vi "Receiver_Example - 2 Channel - Experiment_17.vi"() -> ()   [LabVIEW 2022 SP3]
panel:
  out "SNR dB LP":dbl
  out "SNR dB HP":dbl
  out "size(s) 4":i32
  out "size(s) 3":i32
  out "size(s) 2":i32
  out "x*y":i32
  out "Payload_LP":i32=720
  out "Payload_HP":i32=720
  out "size(s)":i32
  in  "stop":bool
  out "BER LP3":dbl
  out "BER HP3":dbl
  out "Inst. BER LP - CH1":dbl format="%#_4g"
  out "OutputHPCH0":i8[](array[numeric])
  out "BER 16QAM":dbl
  out "LP - CH0":dbl format="%#_4g"
  out "Numeric":i32
  out "HP - CH0":dbl format="%#_4g"
  out "x = 0?":bool
  out "iterationsIM":dbl
  in  "State":i32
  in  "Counter":dbl
  in  "Tab Control 3":enum32{"OFDM - 4QAM", "16QAM"}(tab)
  in  "Switch mode":bool
  in  "Tab Control":T1(tab)
  in  "USRP ControledParameters":T2={"Active Antenna"="RX2", "Gain (dB)"=20.0, "Carrier Frequency"=2400000000.0, "IQ Rate"=2000000.0, "Active channels"="0,1"} {"IQ Rate" format="%#_6p"; "Carrier Frequency" format="%#_6p"; "Gain (dB)" format="%#_6f"}
  in  "Device selection":refnum<k15>="RIO0"
  in  "Trigger level":dbl=0.01 format="%f"
  out "CH0 - HP":T3
  out "CH1 - HP":T3
  out "SIG valid? - CH1":bool
  out "SIG valid? - CH0":bool
  out "Frequency offset - CH1":dbl
  out "Frequency offset - CH0":dbl
  out "Coerced Parameters":T4={"IQ Rate"=100000.0, "Carrier  Freq."=100000.0, "Gain"=0.0} {"Gain" format="%#_6f"; "Carrier  Freq." format="%#_6p"; "IQ Rate" format="%#_6p"}
  out "Error out":errorcluster
  out "CH0 - LP":T3
  out "CH1 - LP":T3
  out "Inst. BER HP - CH0":dbl format="%#_4g"
  out "Acc. BER HP - CH0":dbl format="%#_4g"
  out "Acum. Err HP - CH0":dbl
  out "No. Bits HP - CH0":dbl
  out "Acc. BER LP - CH0":dbl format="%#_4g"
  out "Inst. BER - CH1":dbl format="%#_4g"
  out "Inst. BER LP - CH0":dbl format="%#_4g"
  out "No. Bits - CH1":dbl
  out "No. Bits LP - CH0":dbl
  out "Acum. Err - CH1":dbl
  out "Acum. Err LP - CH0":dbl
  in  "Record BER":bool
  in  "Refresh Button":bool
  out "Acc. BER - CH1":dbl format="%#_4g"
  in  "Boolean 2":bool
  in  "Expected message HP - CH0":string="Critical Dataaaaa\nCritical Dataaaaa\nCritical Dataaaaa\nCritical Dataaaaa\nCritical Dataaaaa"
  out "Expected message HP Detected CH0":string="Non Critical Data\nNon Critical Data\nNon Critical Data\nNon Critical Data\nNon Critical Data"
  in  "Boolean 3":bool
  in  "Boolean":bool
  out "Expected message HP Detected CH1":string="Non Critical Data\nNon Critical Data\nNon Critical Data\nNon Critical Data\nNon Critical Data"
  out "Expected message LP Detected CH0":string="Non Critical Data\nNon Critical Data\nNon Critical Data\nNon Critical Data\nNon Critical Data"
  in  "Expected message - CH1":string="Critical Dataaaaa\nCritical Dataaaaa\nCritical Dataaaaa\nCritical Dataaaaa\nCritical Dataaaaa"
  in  "Expected message LP - CH0":string="Non Critical Data\nNon Critical Data\nNon Critical Data\nNon Critical Data\nNon Critical Data"
  in  "Boolean 5":bool
  in  "Expected message LP - CH1":string="Non Critical Data\nNon Critical Data\nNon Critical Data\nNon Critical Data\nNon Critical Data"
  out "Expected message LP Detected CH1":string="Non Critical Data\nNon Critical Data\nNon Critical Data\nNon Critical Data\nNon Critical Data"
  in  "High-Power Window Size":dbl=15.0 format="%#_6p"
  in  "Low-Power Window Size - CH0":dbl=15.0 format="%#_6p"
  in  "Channel":bool
  in  "Expected message HP - CH0 2":string="Critical Dataaaaa\nCritical Dataaaaa\nCritical Dataaaaa\nCritical Dataaaaa\nCritical Dataaaaa\nNon Critical Data\nNon Critical Data\nNon Critical Data\nNon Critical Data\nNon Critical Data"
  in  "Tab Control 2":enum32{"1 Channel", "2 Channel"}(tab)
  in  "Save data 1 channel":bool
  out "Constellation Map 1 Channel":cdb[](graph)
  out "Low-Power BER - 1 Channel":dbl(graph)
  out "High-Power BER - 1 Channel":dbl(graph)
  out "High-Power Decoded message - 1 Channel":string
  out "Low-Power Decoded message - 1 Channel":string
  out "Low-Power Decoded message - CH0":string
  out "Decoded message - CH1":string
  out "Constellation Map 2 Channel":cluster{"Constellation":cdb[]}[](graph)
  out "Low-Power BER - 2 Channels":T5(graph)
  out "High-Power BER":T6(graph)
  out "High-Power Decoded message - CH0":string
  out "Low-Power Decoded message - CH1":string
  out "CH1 2":bool
  out "CH0 2":bool
  in  "Save data 2 channels":bool
  in  "Color Box 3":u32(colorbox)=11025761
  in  "Color Box 4":u32(colorbox)=7377308
  out "SNR dB":dbl
  in  "Save data":bool
  out "Expected message  HP  Detected 2":string="Critical Dataaaaa\nCritical Dataaaaa\nCritical Dataaaaa\nCritical Dataaaaa\nCritical Dataaaaa"
  in  "Boolean 4":bool
  in  "High-Power Window Size 2":dbl=15.0 format="%#_6p"
  out "High-Power Instantaneous BER Graph 2":u8(slide) scale=0.0..100.0
  out "High-Power BER Graph 2":dbl(graph)
  out "No. Bits HP 2":dbl
  out "Acc. BER  HP 2":dbl format="%#_4g"
  out "Acum. Err HP 2":dbl
  out "Inst. BER HP 2":dbl format="%#_4g"
  in  "Expected message 2 HP 2":string="Critical Dataaaaa\nCritical Dataaaaa\nCritical Dataaaaa\nCritical Dataaaaa\nCritical Dataaaaa"
  out "High-Power Decoded Message 2":string
  in  "Record BER 2":bool
  out "Constellation Map 2":cdb[](graph)
  out "Frequency offset 2":dbl
  out "SIG valid? 2":bool
  in  "Refresh Button 2":bool
  out "Error out 2":errorcluster
  in  "error in (no error)":errorcluster
  # "OFDM Superposition Coded Receiver"
  # "Superposition coded\n(criticality-aware)"
  # "Single stream\n(criticality-agnostic)"
  # "1 Channel"
  # "2 Channel"
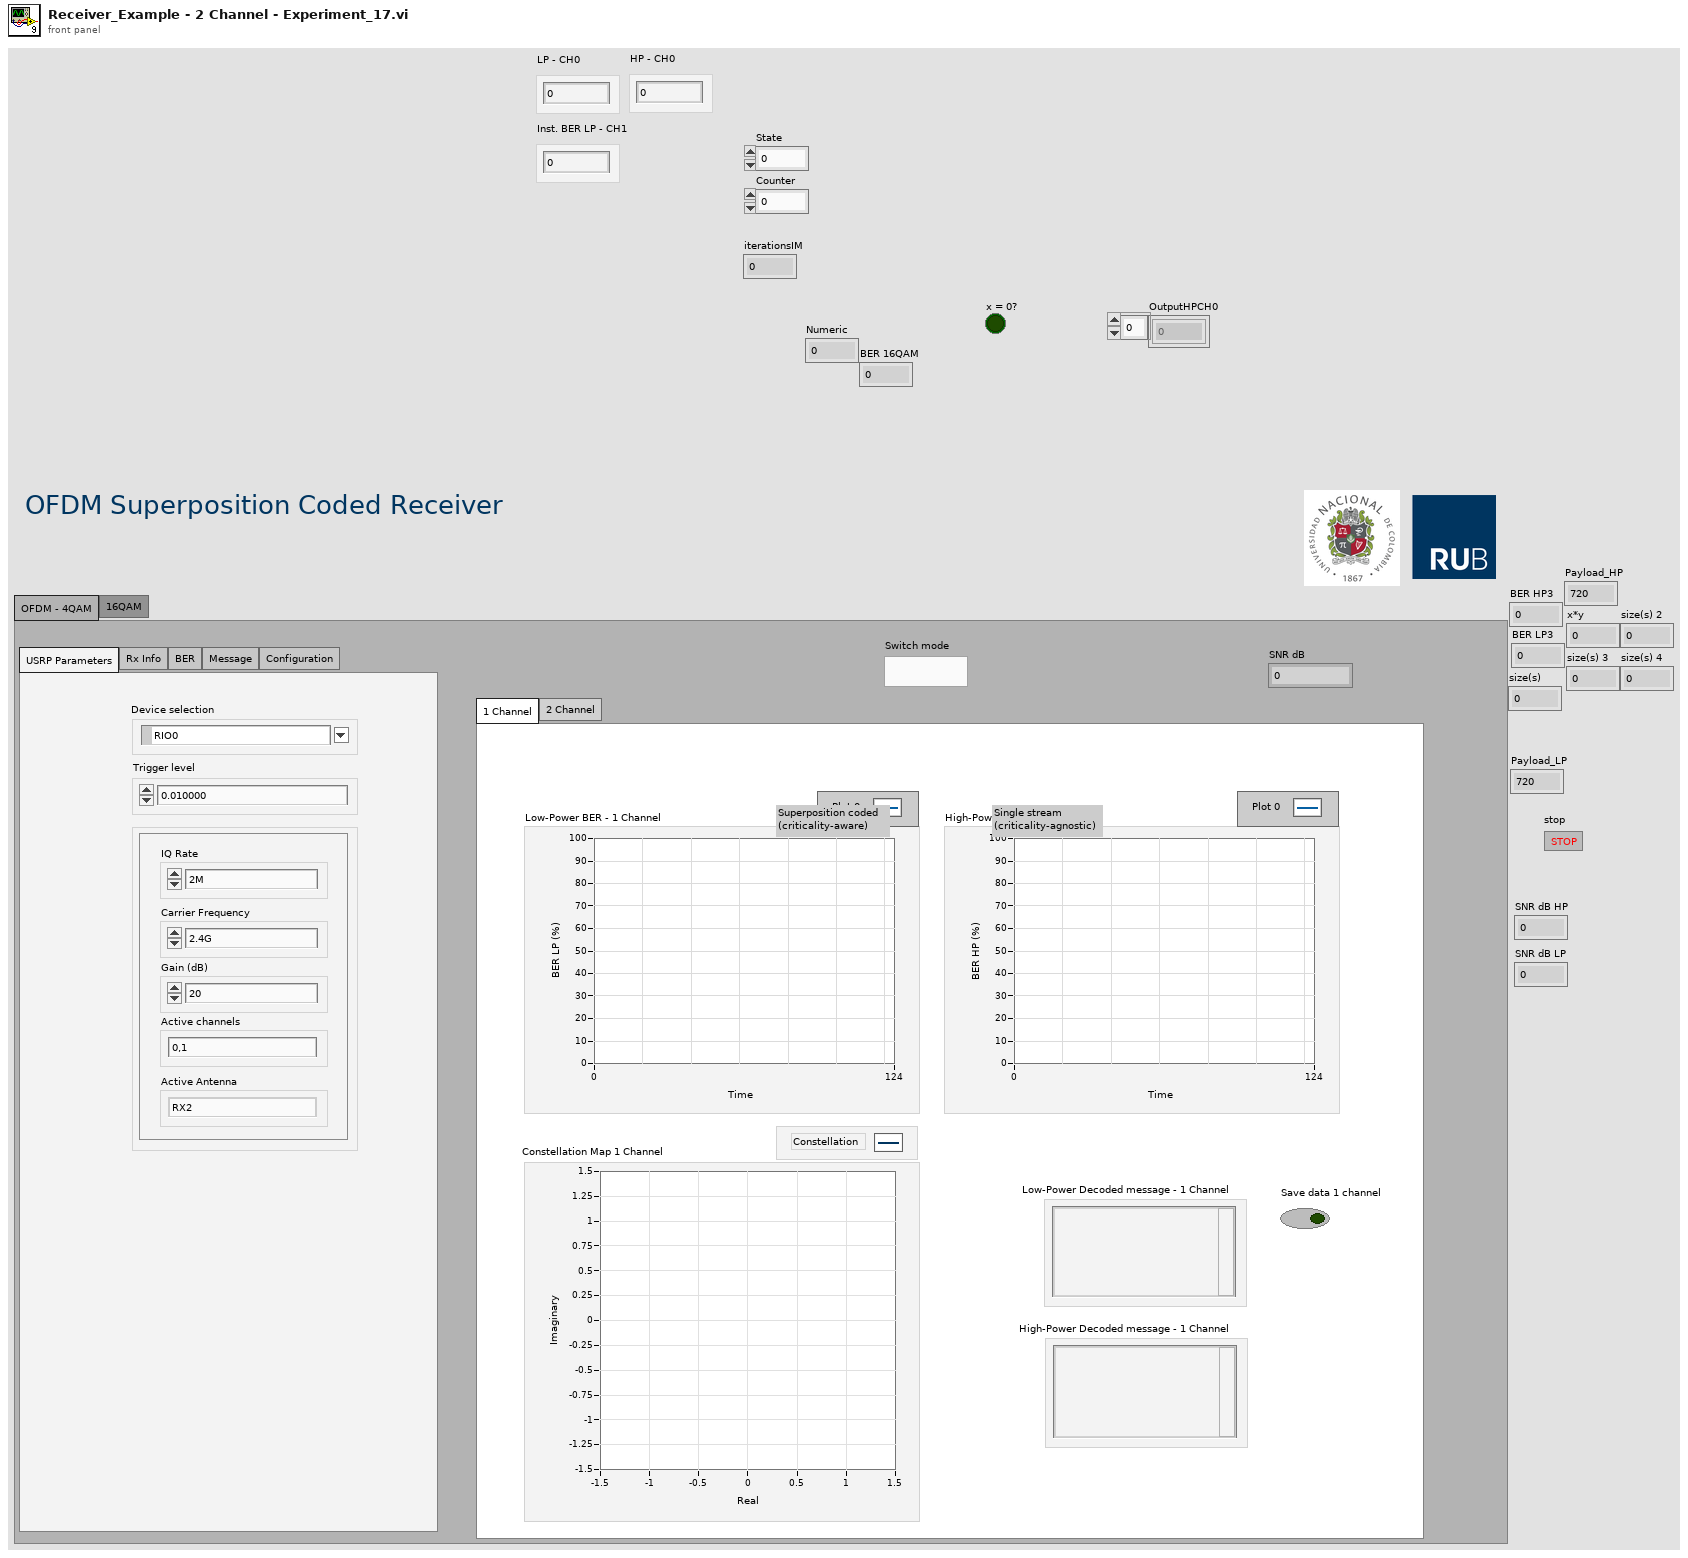
[diagram p1: front panel]
types:
  T1 = enum32{"USRP Parameters", "Rx Info", "BER", "Message", "Configuration"}
  T2 = cluster{"Active Antenna":string, "Gain (dB)":dbl, "Carrier Frequency":dbl, "IQ Rate":dbl, "Active channels":string}
  T3 = cluster{"Modulation type":enum16{"QPSK(4QAM)", "64QAM", "16QAM", "BPSK"}, "BCC rate (k/n)":enum16{"1/2", "2/3", "3/4"}}
  T4 = cluster{"IQ Rate":dbl, "Carrier  Freq.":dbl, "Gain":dbl}
  T5 = cluster{"Graph Instantaneous BER":dbl, "Graph Instantaneous BER":dbl, "Graph Instantaneous BER":dbl}
  T6 = cluster{"Graph Instantaneous BER":dbl, "Graph Instantaneous BER":dbl, "Inst. BER - CH1":dbl}
  T7 = enum16{"open", "replace", "create", "open or create", "replace or create", "replace or create with confirmation"}
  T8 = cluster{"coerced IQ rate":dbl, "coerced carrier frequency":dbl, "coerced gain":dbl}
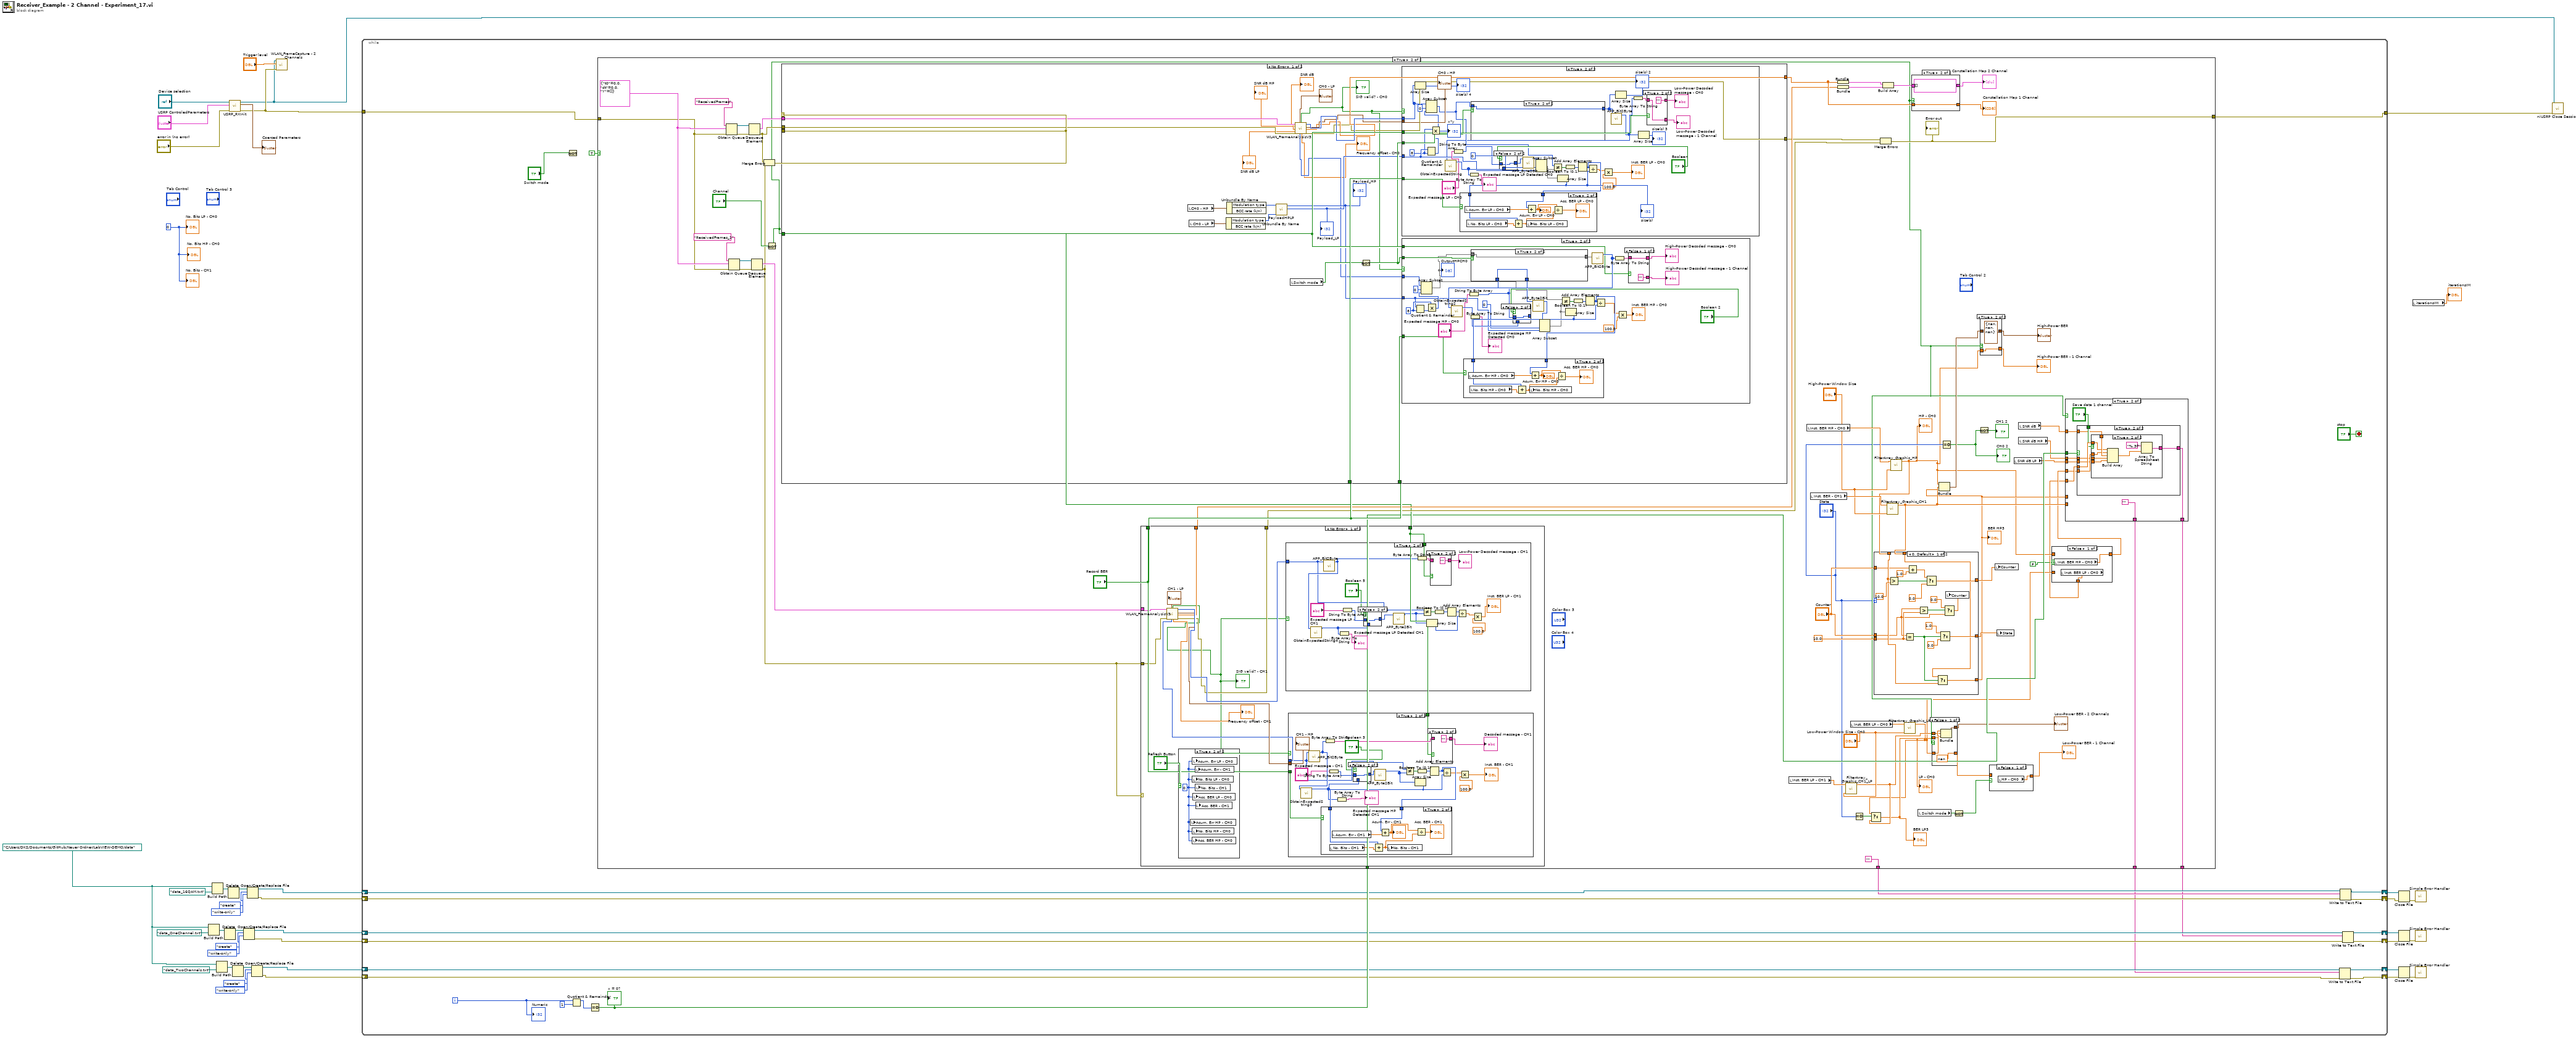
[diagram p0: block diagram]
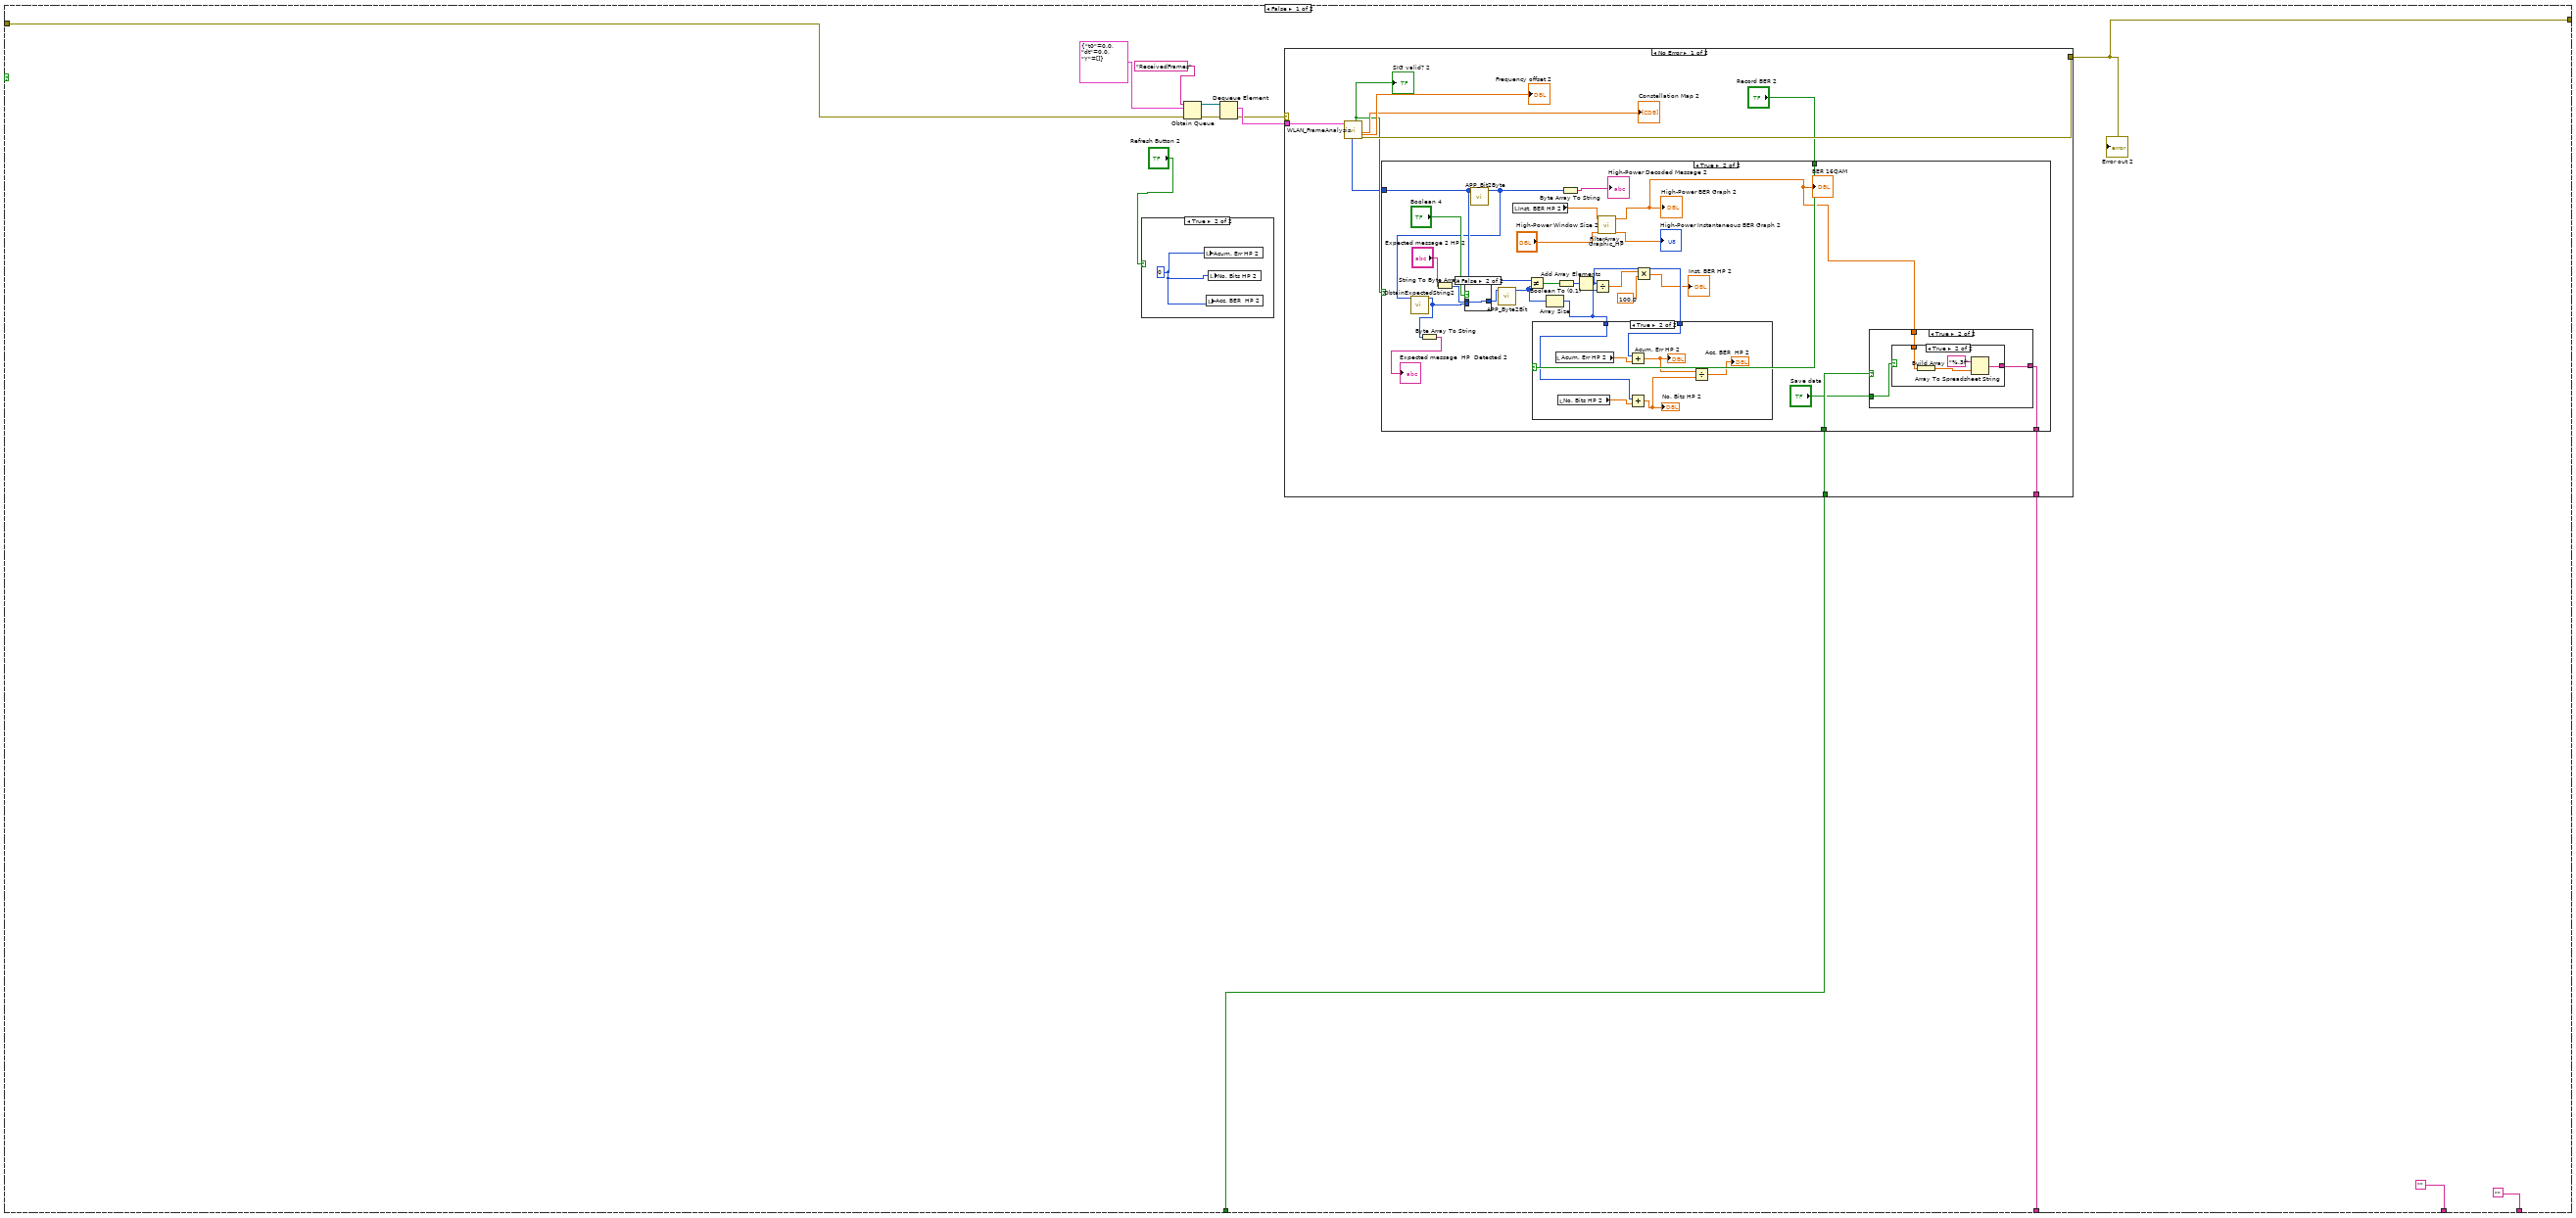
[diagram p2: hidden frame]
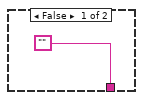
[diagram p4: hidden frame]
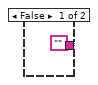
[diagram p5: hidden frame]
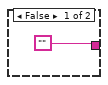
[diagram p6: hidden frame]
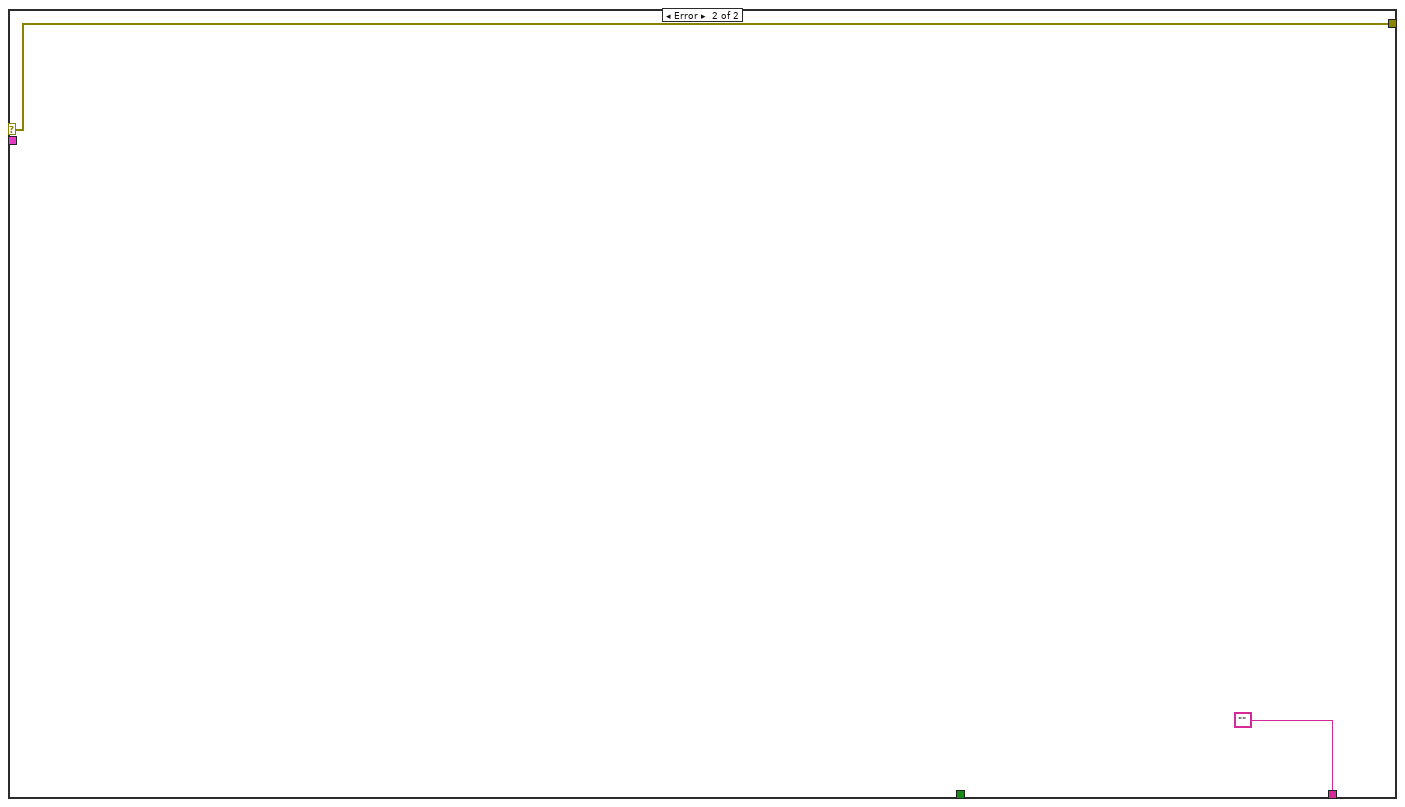
[diagram p9: hidden frame]
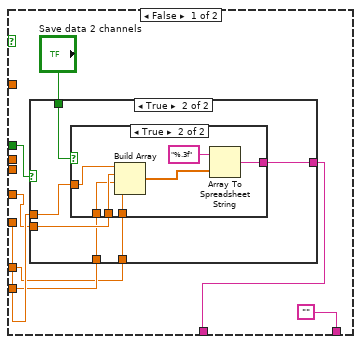
[diagram p12: hidden frame]
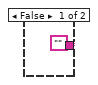
[diagram p13: hidden frame]
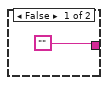
[diagram p14: hidden frame]
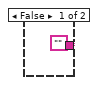
[diagram p15: hidden frame]
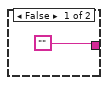
[diagram p16: hidden frame]
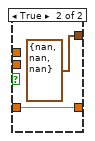
[diagram p17: hidden frame]
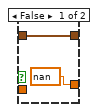
[diagram p18: hidden frame]
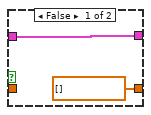
[diagram p19: hidden frame]
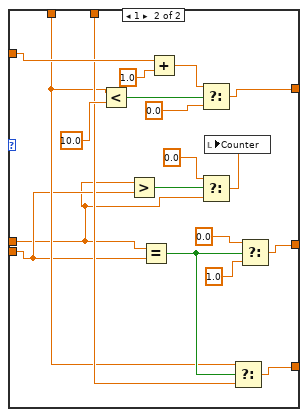
[diagram p20: hidden frame]
diagram:
  w11 = path "C:/Users/DKS/Documents/GitHub/Neuer Ordner/LabVIEW-DEMO/data"
  w33 = 0
  n1 = Build Path(base path=w11, name or relative path=path "data_OneChannel.txt" ("default name")) -> (appended path=w21:path)
  n2 = Build Path(base path=w11, name or relative path=path "data_16QAM.txt" ("default name")) -> (appended path=w31:path)
  n3 = Build Path(base path=w11, name or relative path=path "data_TwoChannels.txt" ("default name")) -> (appended path=w16:path)
  n4 = Delete(path (use dialog)=w21) -> (deleted path=w20:path)  [unwired: 4 in, 2 out]
  n5 = Delete(path (use dialog)=w31) -> (deleted path=w30:path)  [unwired: 4 in, 2 out]
  n6 = call "USRP_RXInit.vi"("device names"="Device selection", "USRP ControledParameters"="USRP ControledParameters", "error in (no error)"="error in (no error)") -> ("session handle out"=w36:refnum<k15>, "USRP CoercedParamters"=→"Coerced Parameters":T8, "error out"=w39:errorcluster)  [unwired: 5 in]
  n7 = Delete(path (use dialog)=w16) -> (deleted path=w15:path)  [unwired: 4 in, 2 out]
  n8 = Open/Create/Replace File(file path (use dialog)=w20, operation (0:open)=T7."create", access (0:read/write)=enum16{"read/write", "read-only", "write-only"}."write-only") -> (refnum out=w8:refnum<file>, error out=w7:errorcluster)  [unwired: 1 in, 3 out]
  n9 = Open/Create/Replace File(file path (use dialog)=w30, operation (0:open)=T7."create", access (0:read/write)=enum16{"read/write", "read-only", "write-only"}."write-only") -> (refnum out=w24:refnum<file>, error out=w25:errorcluster)  [unwired: 1 in, 3 out]
  n10 = Open/Create/Replace File(file path (use dialog)=w15, operation (0:open)=T7."create", access (0:read/write)=enum16{"read/write", "read-only", "write-only"}."write-only") -> (refnum out=w6:refnum<file>, error out=w5:errorcluster)  [unwired: 1 in, 3 out]
  n11 = call "WLAN_FrameCapture - 2 Channels.vi"("error in (no error)"=w39, "Trigger level"="Trigger level", "session handle"=w36) -> ()  [unwired: 8 in]
  n12 = while {
    tunnel: w39 -> [w65]
    tunnel: [w64] -> w37
    shift-right: [w60] -> w23
    shift-left: w25 -> [w58]
    shift-right: [w59] -> w22
    shift-left: w24 -> [w57]
    shift-right: [w54] -> w4
    shift-left: w8 -> [w55]
    shift-right: [w52] -> w3
    shift-left: w7 -> [w53]
    shift-right: [w48] -> w2
    shift-left: w6 -> [w51]
    shift-right: [w49] -> w1
    shift-left: w5 -> [w50]
    i -> [w45]
    stop <- "stop" stop-if-true
    n13 = Not(x="Switch mode") -> ()  [unwired: 1 out]
    n14 = Quotient & Remainder(x=w45, y=1) -> (x-y*floor(x/y)=w62:i32)  [unwired: 1 out]
    n15 = Equal To 0?(x=w62) -> (x = 0?=w61:bool)
    "x = 0?" <- w61
    n16 = case shown="True" TRUE {
      tunnel: w65 -> [w71 w164]
      tunnel: [w70 w163] -> w64
      tunnel: w61 -> [w69 w159]
      tunnel: [w68 ""] -> w56
      tunnel: ["" w158] -> w47
      tunnel: ["" w156] -> w46
      frame False {
        n17 = case shown="True" "Refresh Button 2" {
          frame False {
          }
          frame True {
            w79 = 0
            n18 = local write "Acum. Err HP 2"(w79) -> ()
            n19 = local write "Acc. BER  HP 2"(w79) -> ()
            n20 = local write "No. Bits HP 2"(w79) -> ()
          }
        }
        n21 = Obtain Queue(name (unnamed)="ReceivedFrames", element data type=cluster{"t0":dbl, "dt":dbl, "Y":cdb[]} {"t0"=0.0, "dt"=0.0, "Y"=[]} ("data"), error in (no error)=w71) -> (queue out=w72:refnum<queue>, error out=w75:errorcluster)  [unwired: 2 in, 1 out]
        n22 = Dequeue Element(queue=w72, error in (no error)=w75) -> (element=w74:cluster{"t0":dbl, "dt":dbl, "Y":cdb[]}, error out=w73:errorcluster)  [unwired: 1 in, 2 out]
        n23 = case shown="No Error" w73 {
          selector: w73 -> [_ w134]
          tunnel: w74 -> [w87 _]
          tunnel: [w88 w134] -> w70
          tunnel: w69 -> [w81 _]
          tunnel: [w80 ""] -> w68
          frame No Error {
            n24 = call "WLAN_FrameAnalysis.vi"("input cluster"=w87) -> ("error out"=w88:errorcluster, "Constellation"=→"Constellation Map 2":cdb[], "Frequency offset"=→"Frequency offset 2":dbl, "SIG valid?"=w83:bool, "outputbitsHP"=w82:i8[])  [unwired: 4 in, 2 out]
            "SIG valid? 2" <- w83
            n25 = case shown="True" w83 {
              tunnel: "Record BER 2" -> [_ w108]
              tunnel: w82 -> [_ w103]
              tunnel: w81 -> [_ w93]
              tunnel: ["" w91] -> w80
              frame False {
              }
              frame True {
                n26 = String To Byte Array(string="Expected message 2 HP 2") -> (unsigned byte array=w101:u8[])
                n27 = call "APP_Bit2Byte.vi"("input bit stream"=w103) -> ("output byte stream"=w97:u8[])  [unwired: 10 in]
                n28 = call "ObtainExpectedString2.vi"("Array"=w97) -> ("detectedMessage"=w99:i8[])  [unwired: 9 in]
                n29 = Byte Array To String(unsigned byte array=w99) -> (string=→"Expected message  HP  Detected 2":string)
                n30 = case shown="False" "Boolean 4" {
                  tunnel: [w124 w125] -> w102
                  tunnel: w101 -> [_ w125]
                  tunnel: w99 -> [w124 _]
                  frame True {
                  }
                  frame False {
                  }
                }
                n31 = call "APP_Byte2Bit.vi"("input byte stream"=w102) -> ("output bit stream"=w104:i8[])  [unwired: 10 in]
                n32 = local read "Inst. BER HP 2"() -> (w107:dbl)
                n33 = Not Equal?(x=w103, y=w104) -> (x != y?=w112:bool[])
                n34 = Array Size(array=w104) -> (size(s)=w109:i32)
                n35 = Boolean To (0,1)(Boolean=w112) -> (0, 1=w111:i16[])
                n36 = Byte Array To String(unsigned byte array=w97) -> (string=→"High-Power Decoded Message 2":string)
                n37 = Add Array Elements(numeric array=w111) -> (sum=w110:i16)
                n38 = case shown="True" w108 {
                  tunnel: w110 -> [_ w131]
                  tunnel: w109 -> [_ w126]
                  frame False {
                  }
                  frame True {
                    n39 = local read "Acum. Err HP 2"() -> (w132:dbl)
                    n40 = local read "No. Bits HP 2"() -> (w128:dbl)
                    n41 = Add(x=w131, y=w132) -> (x+y=w130:dbl)
                    "Acum. Err HP 2" <- w130
                    n42 = Add(x=w126, y=w128) -> (x+y=w127:dbl)
                    "No. Bits HP 2" <- w127
                    n43 = Divide(x=w130, y=w127) -> (x/y=→"Acc. BER  HP 2":dbl)
                  }
                }
                n44 = Divide(x=w110, y=w109) -> (x/y=w96:dbl)
                n45 = call "FilterArray_Graphic_HP.vi"("Window Size"="High-Power Window Size 2", "Instantaneous BER"=w107) -> ("Slide Bar"=→"High-Power Instantaneous BER Graph 2":dbl, "Graph Instantaneous BER"=w90:dbl)  [unwired: 4 in]
                "High-Power BER Graph 2" <- w90
                "BER 16QAM" <- w90
                n46 = Multiply(x=w96, y=100.0) -> (x*y=→"Inst. BER HP 2":dbl)
                n47 = case shown="True" w93 {
                  tunnel: ["" w118] -> w91
                  tunnel: w90 -> [_ w117]
                  tunnel: "Save data" -> [_ w116]
                  frame False {
                  }
                  frame True {
                    n48 = case shown="True" w116 {
                      tunnel: ["" w121] -> w118
                      tunnel: w117 -> [_ w120]
                      frame False {
                      }
                      frame True {
                        n49 = Build Array(w120) -> (w123:dbl[])
                        n50 = Array To Spreadsheet String(array=w123, 3:"%.3f") -> (spreadsheet string=w121:string)  [unwired: 1 out]
                      }
                    }
                  }
                }
              }
            }
          }
          frame Error {
          }
        }
        "Error out 2" <- w70
      }
      frame True {
        w198 = cluster{"t0":dbl, "dt":dbl, "Y":cdb[]} {"t0"=0.0, "dt"=0.0, "Y"=[]} ("data")
        n51 = Obtain Queue(name (unnamed)="ReceivedFrames", element data type=w198, error in (no error)=w164) -> (queue out=w165:refnum<queue>, error out=w167:errorcluster)  [unwired: 2 in, 1 out]
        n52 = Obtain Queue(name (unnamed)="ReceivedFrames_1", element data type=w198, error in (no error)=w164) -> (queue out=w169:refnum<queue>, error out=w170:errorcluster)  [unwired: 2 in, 1 out]
        n53 = Dequeue Element(queue=w165, error in (no error)=w167) -> (element=w166:cluster{"t0":dbl, "dt":dbl, "Y":cdb[]}, error out=w173:errorcluster)  [unwired: 1 in, 2 out]
        n54 = Dequeue Element(queue=w169, error in (no error)=w170) -> (element=w175:cluster{"t0":dbl, "dt":dbl, "Y":cdb[]}, error out=w143:errorcluster)  [unwired: 1 in, 2 out]
        n55 = Merge Errors(w173, w143) -> (w172:errorcluster)
        n56 = Not(x="Channel") -> (.not. x?=w160:bool)
        n57 = case shown="No Error" w172 {
          tunnel: w166 -> [w384 _]
          tunnel: w172 -> [_ w517]
          tunnel: w173 -> [w382 _]
          tunnel: [w388 dbl[] []] -> w189
          tunnel: [w387 w517] -> w176
          tunnel: "Record BER" -> [w401 _]
          tunnel: "Record BER" -> [w400 _]
          tunnel: w160 -> [w399 _]
          frame No Error {
            n58 = local read "CH0 - HP"() -> (w394:T3)
            n59 = local read "CH0 - LP"() -> (w393:T3)
            n60 = Unbundle By Name(w393) -> ("Modulation type"=w395:enum16{"QPSK(4QAM)", "64QAM", "16QAM", "BPSK"})  [unwired: 1 out]
            n61 = Unbundle By Name(w394) -> ("Modulation type"=w396:enum16{"QPSK(4QAM)", "64QAM", "16QAM", "BPSK"})  [unwired: 1 out]
            n62 = call "PayloadHPLP.vi"("Modulation type LP"=w395, "Modulation type HP"=w396) -> ("Payload_LP"=w392:i32, "Payload_HP"=w391:i32)  [unwired: 8 in]
            "Payload_HP" <- w391
            "Payload_LP" <- w392
            n63 = local read "Switch mode"() -> (w398:bool)
            n64 = call "WLAN_FrameAnalysisV3.vi"("input cluster"=w384, "error in (no error)"=w382) -> ("SNR dB"=→"SNR dB":dbl, "Modulation parameter LP"=→"CH0 - LP":T3, "outputbitsHP"=w381:i8[], "SIG valid?"=w386:bool, "Frequency offset"=→"Frequency offset - CH0":dbl, "SNR dB HP"=→"SNR dB HP":dbl, "SNR dB LP"=→"SNR dB LP":dbl, "output bits"=w390:i8[], "Modulation parameter"=w389:T3, "Constellation"=w388:cdb[], "error out"=w387:errorcluster)  [unwired: 7 in]
            "SIG valid? - CH0" <- w386
            n65 = Not(x=w398) -> (.not. x?=w397:bool)
            n66 = case shown="True" w386 {
              tunnel: w390 -> [_ w459]
              tunnel: w389 -> [_ w492]
              tunnel: w400 -> [_ w489]
              tunnel: w399 -> [_ w479]
              tunnel: w397 -> [_ w478]
              tunnel: w392 -> [_ w469]
              frame False {
              }
              frame True {
                w465 = 8 ("y")
                n67 = Array Size(array=w459) -> (size(s)=→"size(s) 4":i32)
                n68 = Quotient & Remainder(x=w469, y=w465) -> (floor(x/y)=w466:i32)  [unwired: 1 out]
                n69 = Multiply(x=w465, y=w466) -> (x*y=w464:i32)
                "x*y" <- w464
                n70 = Array Subset(array=w459, index=0, length=w464) -> (w468:i8[])
                n71 = String To Byte Array(string="Expected message LP - CH0") -> (unsigned byte array=w472:u8[])
                n72 = case shown="True" w478 {
                  tunnel: w468 -> [_ w502]
                  tunnel: [w500 w502] -> w463
                  frame False {
                    n73 = local read "OutputHPCH0"() -> (w499:i8[])
                    n74 = Array Size(array=w499) -> (size(s)=w498:i32)
                    n75 = Divide(x=w498, y=2) -> (x/y=w495:dbl)
                    n76 = Add(x=4.0, y=w495) -> (x+y=w497:dbl)
                    n77 = Subtract(x=w495, y=5.0) -> (x-y=w493:dbl)
                    n78 = Array Subset(array=w499, index=w497, length=w493) -> (w500:i8[])
                  }
                  frame True {
                  }
                }
                n79 = call "APP_Bit2Byte.vi"("input bit stream"=w463) -> ("output byte stream"=w461:u8[])  [unwired: 10 in]
                n80 = call "ObtainExpectedString.vi"("Array"=w461) -> ("detectedMessage"=w484:i8[])  [unwired: 9 in]
                n81 = Byte Array To String(unsigned byte array=w484) -> (string=→"Expected message LP Detected CH0":string)
                n82 = case shown="False" "Boolean" {
                  tunnel: [w507 w508] -> w473
                  tunnel: w472 -> [_ w508]
                  tunnel: w484 -> [w507 _]
                  frame True {
                  }
                  frame False {
                  }
                }
                n83 = call "APP_Byte2Bit.vi"("input byte stream"=w473) -> ("output bit stream"=w471:i8[])  [unwired: 10 in]
                n84 = Array Subset(array=w471, index=0, length=w469) -> (w470:i8[])
                n85 = Not Equal?(x=w468, y=w470) -> (x != y?=w490:bool[])
                n86 = Array Size(array=w470) -> (size(s)=w488:i32)
                "size(s)" <- w488
                n87 = Boolean To (0,1)(Boolean=w490) -> (0, 1=w491:i16[])
                n88 = Add Array Elements(numeric array=w491) -> (sum=w487:i16)
                n89 = case shown="True" w489 {
                  tunnel: w488 -> [_ w514]
                  tunnel: w487 -> [_ w512]
                  frame False {
                  }
                  frame True {
                    n90 = local read "Acum. Err LP - CH0"() -> (w513:dbl)
                    n91 = local read "No. Bits LP - CH0"() -> (w515:dbl)
                    n92 = Add(x=w514, y=w515) -> (x+y=w511:dbl)
                    n93 = Add(x=w512, y=w513) -> (x+y=w510:dbl)
                    "Acum. Err LP - CH0" <- w510
                    n94 = local write "No. Bits LP - CH0"(w511) -> ()
                    n95 = Divide(x=w510, y=w511) -> (x/y=→"Acc. BER LP - CH0":dbl)
                  }
                }
                n96 = Divide(x=w487, y=w488) -> (x/y=w486:dbl)
                n97 = Multiply(x=w486, y=100.0) -> (x*y=→"Inst. BER LP - CH0":dbl)
                n98 = Array Size(array=w463) -> (size(s)=→"size(s) 2":i32)
                n99 = Byte Array To String(unsigned byte array=w461) -> (string=w482:string)
                n100 = Array Size(array=w461) -> (size(s)=→"size(s) 3":i32)
                n101 = case shown="True" w479 {
                  tunnel: w482 -> [w504 w506]
                  tunnel: ["" ("string") w506] -> w481
                  tunnel: [w504 "" ("string")] -> w480
                  frame False {
                  }
                  frame True {
                  }
                }
                "Low-Power Decoded message - CH0" <- w480
                "Low-Power Decoded message - 1 Channel" <- w481
                "CH0 - HP" <- w492
              }
            }
            n102 = case shown="True" w386 {
              tunnel: w381 -> [_ w403]
              tunnel: w401 -> [_ w430]
              tunnel: w399 -> [_ w419]
              tunnel: w397 -> [_ w417]
              tunnel: w391 -> [_ w404]
              frame False {
              }
              frame True {
                w406 = 8 ("y")
                n103 = Quotient & Remainder(x=w404, y=w406) -> (floor(x/y)=w407:i32)  [unwired: 1 out]
                n104 = Multiply(x=w406, y=w407) -> (x*y=w405:i32)
                n105 = Array Subset(array=w403, index=0, length=w405) -> (w402:i8[])
                "OutputHPCH0" <- w402
                n106 = String To Byte Array(string="Expected message HP - CH0") -> (unsigned byte array=w411:u8[])
                n107 = case shown="True" w417 {
                  tunnel: w402 -> [w440 w444]
                  tunnel: [w441 w444] -> w418
                  tunnel: [w433 w443] -> w416
                  tunnel: w411 -> [_ w443]
                  frame False {
                    n108 = Array Size(array=w440) -> (size(s)=w437:i32)
                    n109 = Divide(x=w437, y=2) -> (x/y=w436:dbl)
                    n110 = Subtract(x=w436, y=5) -> (x-y=w438:dbl)
                    n111 = Array Subset(array=w440, index=0, length=w438) -> (w441:i8[])
                    n112 = String To Byte Array(string="Expected message HP - CH0 2") -> (unsigned byte array=w433:u8[])
                  }
                  frame True {
                  }
                }
                n113 = call "APP_Byte2Bit.vi"("input byte stream"=w416) -> ("output bit stream"=w410:i8[])  [unwired: 10 in]
                n114 = Array Subset(array=w410, index=0, length=w404) -> (w409:i8[])
                n115 = Not Equal?(x=w402, y=w409) -> (x != y?=w431:bool[])
                n116 = Array Size(array=w409) -> (size(s)=w429:i32)
                n117 = Boolean To (0,1)(Boolean=w431) -> (0, 1=w432:i16[])
                n118 = Add Array Elements(numeric array=w432) -> (sum=w428:i16)
                n119 = case shown="True" w430 {
                  tunnel: w429 -> [_ w456]
                  tunnel: w428 -> [_ w454]
                  frame False {
                  }
                  frame True {
                    n120 = local read "Acum. Err HP - CH0"() -> (w455:dbl)
                    n121 = local read "No. Bits HP - CH0"() -> (w457:dbl)
                    n122 = Add(x=w456, y=w457) -> (x+y=w453:dbl)
                    n123 = local write "No. Bits HP - CH0"(w453) -> ()
                    n124 = Add(x=w454, y=w455) -> (x+y=w452:dbl)
                    "Acum. Err HP - CH0" <- w452
                    n125 = Divide(x=w452, y=w453) -> (x/y=→"Acc. BER HP - CH0":dbl)
                  }
                }
                n126 = call "APP_Bit2Byte.vi"("input bit stream"=w418) -> ("output byte stream"=w425:u8[])  [unwired: 10 in]
                n127 = call "ObtainExpectedString2.vi"("Array"=w425) -> ("detectedMessage"=w424:i8[])  [unwired: 9 in]
                n128 = Byte Array To String(unsigned byte array=w424) -> (string=→"Expected message HP Detected CH0":string)
                n129 = case shown="False" "Boolean 2" {
                  tunnel: [w449 w450] -> _
                  tunnel: w411 -> [_ w450]
                  tunnel: w424 -> [w449 _]
                  frame True {
                  }
                  frame False {
                  }
                }
                n130 = Divide(x=w428, y=w429) -> (x/y=w427:dbl)
                n131 = Byte Array To String(unsigned byte array=w425) -> (string=w420:string)
                n132 = Multiply(x=w427, y=100.0) -> (x*y=→"Inst. BER HP - CH0":dbl)
                n133 = case shown="False" w419 {
                  tunnel: w420 -> [w446 w448]
                  tunnel: ["" ("string") w448] -> w421
                  tunnel: [w446 "" ("string")] -> w422
                  frame False {
                  }
                  frame True {
                  }
                }
                "High-Power Decoded message - CH0" <- w422
                "High-Power Decoded message - 1 Channel" <- w421
              }
            }
          }
          frame Error {
          }
        }
        n134 = case shown="No Error" w143 {
          tunnel: w175 -> [w309 _]
          tunnel: "Record BER" -> [w318 _]
          tunnel: [w313 w376] -> w177
          tunnel: [w314 dbl[] []] -> w178
          tunnel: w160 -> [w317 _]
          tunnel: w143 -> [w310 w376]
          frame No Error {
            n135 = call "WLAN_FrameAnalysisV3.vi"("input cluster"=w309, "error in (no error)"=w310) -> ("Modulation parameter LP"=→"CH1 - LP":T3, "outputbitsHP"=w311:i8[], "SIG valid?"=w308:bool, "Frequency offset"=→"Frequency offset - CH1":dbl, "output bits"=w316:i8[], "Modulation parameter"=w315:T3, "Constellation"=w314:cdb[], "error out"=w313:errorcluster)  [unwired: 7 in, 3 out]
            "SIG valid? - CH1" <- w308
            n136 = case shown="True" "Refresh Button" {
              frame False {
              }
              frame True {
                w343 = 0
                n137 = local write "Acum. Err HP - CH0"(w343) -> ()
                n138 = local write "Acc. BER HP - CH0"(w343) -> ()
                n139 = local write "Acum. Err LP - CH0"(w343) -> ()
                n140 = local write "No. Bits LP - CH0"(w343) -> ()
                n141 = local write "No. Bits HP - CH0"(w343) -> ()
                n142 = local write "Acc. BER LP - CH0"(w343) -> ()
                n143 = local write "Acum. Err - CH1"(w343) -> ()
                n144 = local write "No. Bits - CH1"(w343) -> ()
                n145 = local write "Acc. BER - CH1"(w343) -> ()
              }
            }
            n146 = case shown="True" w308 {
              tunnel: w316 -> [_ w321]
              tunnel: w317 -> [_ w336]
              frame False {
              }
              frame True {
                n147 = call "APP_Bit2Byte.vi"("input bit stream"=w321) -> ("output byte stream"=w331:u8[])  [unwired: 10 in]
                n148 = call "ObtainExpectedString4.vi"("Array"=w331) -> ("detectedMessage"=w332:i8[])  [unwired: 9 in]
                n149 = Byte Array To String(unsigned byte array=w332) -> (string=→"Expected message LP Detected CH1":string)
                n150 = String To Byte Array(string="Expected message LP - CH1") -> (unsigned byte array=w335:u8[])
                n151 = case shown="False" "Boolean 5" {
                  tunnel: [w339 w340] -> w330
                  tunnel: w335 -> [_ w340]
                  tunnel: w332 -> [w339 _]
                  frame True {
                  }
                  frame False {
                  }
                }
                n152 = call "APP_Byte2Bit.vi"("input byte stream"=w330) -> ("output bit stream"=w322:i8[])  [unwired: 10 in]
                n153 = Byte Array To String(unsigned byte array=w331) -> (string=w338:string)
                n154 = Not Equal?(x=w321, y=w322) -> (x != y?=w328:bool[])
                n155 = Array Size(array=w322) -> (size(s)=w327:i32)
                n156 = case shown="True" w336 {
                  tunnel: w338 -> [w341 _]
                  tunnel: [w341 "" ("string")] -> w337
                  frame False {
                  }
                  frame True {
                  }
                }
                "Low-Power Decoded message - CH1" <- w337
                n157 = Boolean To (0,1)(Boolean=w328) -> (0, 1=w329:i16[])
                n158 = Add Array Elements(numeric array=w329) -> (sum=w326:i16)
                n159 = Divide(x=w326, y=w327) -> (x/y=w325:dbl)
                n160 = Multiply(x=w325, y=100.0) -> (x*y=→"Inst. BER LP - CH1":dbl)
              }
            }
            n161 = case shown="True" w308 {
              tunnel: w311 -> [_ w352]
              tunnel: w315 -> [_ w364]
              tunnel: w318 -> [_ w350]
              tunnel: w317 -> [_ w347]
              frame False {
              }
              frame True {
                n162 = call "APP_Bit2Byte.vi"("input bit stream"=w352) -> ("output byte stream"=w354:u8[])  [unwired: 10 in]
                n163 = call "ObtainExpectedString3.vi"("Array"=w354) -> ("detectedMessage"=w353:i8[])  [unwired: 9 in]
                n164 = Byte Array To String(unsigned byte array=w354) -> (string=w348:string)
                n165 = String To Byte Array(string="Expected message - CH1") -> (unsigned byte array=w355:u8[])
                n166 = Byte Array To String(unsigned byte array=w353) -> (string=→"Expected message HP Detected CH1":string)
                n167 = case shown="False" "Boolean 3" {
                  tunnel: [w367 w368] -> w357
                  tunnel: w355 -> [_ w368]
                  tunnel: w353 -> [w367 _]
                  frame True {
                  }
                  frame False {
                  }
                }
                n168 = call "APP_Byte2Bit.vi"("input byte stream"=w357) -> ("output bit stream"=w356:i8[])  [unwired: 10 in]
                n169 = Not Equal?(x=w352, y=w356) -> (x != y?=w362:bool[])
                n170 = Array Size(array=w356) -> (size(s)=w361:i32)
                n171 = Boolean To (0,1)(Boolean=w362) -> (0, 1=w363:i16[])
                n172 = Add Array Elements(numeric array=w363) -> (sum=w360:i16)
                n173 = case shown="True" w350 {
                  tunnel: w361 -> [_ w374]
                  tunnel: w360 -> [_ w372]
                  frame False {
                  }
                  frame True {
                    n174 = local read "No. Bits - CH1"() -> (w375:dbl)
                    n175 = local read "Acum. Err - CH1"() -> (w373:dbl)
                    n176 = Add(x=w374, y=w375) -> (x+y=w371:dbl)
                    n177 = Add(x=w372, y=w373) -> (x+y=w370:dbl)
                    "Acum. Err - CH1" <- w370
                    n178 = local write "No. Bits - CH1"(w371) -> ()
                    n179 = Divide(x=w370, y=w371) -> (x/y=→"Acc. BER - CH1":dbl)
                  }
                }
                n180 = case shown="True" w347 {
                  tunnel: w348 -> [w365 _]
                  tunnel: [w365 "" ("string")] -> w349
                  frame False {
                  }
                  frame True {
                  }
                }
                "Decoded message - CH1" <- w349
                n181 = Divide(x=w360, y=w361) -> (x/y=w358:dbl)
                n182 = Multiply(x=w358, y=100.0) -> (x*y=→"Inst. BER - CH1":dbl)
                "CH1 - HP" <- w364
              }
            }
          }
          frame Error {
          }
        }
        n183 = local read "Inst. BER LP - CH1"() -> (w149:dbl)
        n184 = local read "Inst. BER HP - CH0"() -> (w194:dbl)
        n185 = local read "Inst. BER - CH1"() -> (w185:dbl)
        n186 = Bundle("Constellation"=w189) -> (w188:cluster{"Constellation":cdb[]})  [unwired: 1 in]
        n187 = Bundle("Constellation"=w178) -> (w174:cluster{"Constellation":cdb[]})  [unwired: 1 in]
        n188 = call "FilterArray_Graphic_CH1_LP.vi"("Window Size"="Low-Power Window Size - CH0", "Instantaneous BER"=w149) -> ("Graph Instantaneous BER"=w145:dbl)  [unwired: 4 in, 1 out]
        n189 = local read "Inst. BER LP - CH0"() -> (w161:dbl)
        n190 = Equal To 0?(x="State") -> (x = 0?=w147:bool)
        n191 = Merge Errors(w176, w177) -> (w163:errorcluster)
        "Error out" <- w163
        n192 = Build Array(w188, w174) -> (w191:cluster{"Constellation":cdb[]}[])
        n193 = call "FilterArray_Graphic_CH1.vi"("Window Size"="High-Power Window Size", "Instantaneous BER"=w185) -> ("Graph Instantaneous BER"=w157:dbl)  [unwired: 4 in, 1 out]
        n194 = call "FilterArray_Graphic_HP.vi"("Window Size"="High-Power Window Size", "Instantaneous BER"=w194) -> ("Graph Instantaneous BER"=w142:dbl)  [unwired: 4 in, 1 out]
        "HP - CH0" <- w142
        n195 = case shown="0, Default" "State" {
          tunnel: "Counter" -> [w275 w295]
          tunnel: [w282 w298] -> w181
          tunnel: "Counter" -> [w270 w288]
          tunnel: [w279 w297] -> w182
          tunnel: [w277 w296] -> w155
          tunnel: w142 -> [w276 w293]
          tunnel: w157 -> [w274 w294]
          tunnel: 10.0 ("y") -> [w273 w289]
          frame 0, Default {
            n196 = Greater?(x=w276, y=10.0) -> (0:w283:bool)
            n197 = Equal?(x=w270, y=w273) -> (x = y?=w278:bool)
            n198 = Add(x=w275, y=1.0) -> (x+y=w285:dbl)
            n199 = Greater?(x=w270, y=w273) -> (0:w272:bool)
            n200 = Select(t=w285, s=w283, f=0.0) -> (s? t:f=w282:dbl)
            n201 = Select(t=w274, s=w278, f=w276) -> (s? t:f=w277:dbl)
            n202 = Select(t=1.0, s=w278, f=0.0) -> (s? t:f=w279:dbl)
            n203 = Select(t=0.0, s=w272, f=w270) -> (s? t:f=w269:dbl)
            n204 = local write "Counter"(w269) -> ()
          }
          frame 1 {
            n205 = Less?(x=w293, y=10.0) -> (x < y?=w299:bool)
            n206 = Greater?(x=w288, y=w289) -> (0:w291:bool)
            n207 = Equal?(x=w288, y=w289) -> (x = y?=w301:bool)
            n208 = Add(x=w295, y=1.0) -> (x+y=w305:dbl)
            n209 = Select(t=w305, s=w299, f=0.0) -> (s? t:f=w298:dbl)
            n210 = Select(t=0.0, s=w291, f=w288) -> (s? t:f=w292:dbl)
            n211 = local write "Counter"(w292) -> ()
            n212 = Select(t=w293, s=w301, f=w294) -> (s? t:f=w296:dbl)
            n213 = Select(t=0.0, s=w301, f=1.0) -> (s? t:f=w297:dbl)
          }
        }
        "BER HP3" <- w155
        n214 = call "FilterArray_Graphic_LP.vi"("Window Size"="Low-Power Window Size - CH0", "Instantaneous BER"=w161) -> ("Graph Instantaneous BER"=w141:dbl)  [unwired: 4 in, 1 out]
        "LP - CH0" <- w141
        n215 = Select(t=w141, s=w147, f=w145) -> (s? t:f=w144:dbl)
        "BER LP3" <- w144
        n216 = case shown="True" w160 {
          tunnel: [cdb[] [] ("Constellation") w268] -> w190
          tunnel: w189 -> [_ w268]
          tunnel: w191 -> [w266 _]
          tunnel: [w266 cluster{"Constellation":cdb[]}[] []] -> w192
          frame False {
          }
          frame True {
          }
        }
        "Constellation Map 2 Channel" <- w192
        "Constellation Map 1 Channel" <- w190
        n217 = local read "Switch mode"() -> (w154:bool)
        n218 = case shown="False" w160 {
          tunnel: w141 -> [w256 w260]
          tunnel: [nan ("Graph Instantaneous BER") w260] -> w151
          tunnel: [w257 T5 {"Graph Instantaneous BER"=nan, "Graph Instantaneous BER"=nan, "Graph Instantaneous BER"=nan}] -> w152
          tunnel: w145 -> [w255 _]
          tunnel: w144 -> [w254 _]
          frame False {
            n219 = Bundle("Graph Instantaneous BER"=w256, "Graph Instantaneous BER"=w255, "Graph Instantaneous BER"=w254) -> (w257:T5)  [unwired: 1 in]
          }
          frame True {
          }
        }
        "Low-Power BER - 2 Channels" <- w152
        n220 = Bundle("Graph Instantaneous BER"=w142, "Graph Instantaneous BER"=w157, "Graph Instantaneous BER"=w155) -> (w196:T5)  [unwired: 1 in]
        n221 = Equal To 0?(x="State") -> (x = 0?=w187:bool)
        "CH0 2" <- w187
        n222 = Not(x=w154) -> (.not. x?=w153:bool)
        n223 = Not(x=w187) -> (.not. x?=→"CH1 2":bool)
        n224 = case shown="True" w160 {
          tunnel: w142 -> [_ w264]
          tunnel: [nan w264] -> w195
          tunnel: w196 -> [w262 _]
          tunnel: [w262 T5 {"Graph Instantaneous BER"=nan, "Graph Instantaneous BER"=nan, "Graph Instantaneous BER"=nan}] -> w197
          frame False {
          }
          frame True {
          }
        }
        "High-Power BER" <- w197
        "High-Power BER - 1 Channel" <- w195
        n225 = case shown="False" w153 {
          tunnel: w151 -> [_ w204]
          tunnel: [w203 w204] -> w150
          frame False {
            n226 = local read "HP - CH0"() -> (w203:dbl)
          }
          frame True {
          }
        }
        "Low-Power BER - 1 Channel" <- w150
        n227 = local write "Counter"(w181) -> ()
        n228 = local write "State"(w182) -> ()
        n229 = local read "SNR dB LP"() -> (w135:dbl)
        n230 = local read "SNR dB"() -> (w137:dbl)
        n231 = local read "SNR dB HP"() -> (w136:dbl)
        n232 = case shown="False" FALSE {
          tunnel: w142 -> [_ w202]
          tunnel: w141 -> [_ w201]
          tunnel: [w200 w202] -> w140
          tunnel: [w199 w201] -> w139
          frame False {
            n233 = local read "Inst. BER HP - CH0"() -> (w200:dbl)
            n234 = local read "Inst. BER LP - CH0"() -> (w199:dbl)
          }
          frame True {
          }
        }
        n235 = case shown="True" w160 {
          tunnel: w139 -> [w209 w236]
          tunnel: w140 -> [w208 w235]
          tunnel: w159 -> [w211 w234]
          tunnel: ["" w232] -> w158
          tunnel: w157 -> [w207 _]
          tunnel: w155 -> [w206 _]
          tunnel: [w205 ""] -> w156
          tunnel: w137 -> [_ w230]
          tunnel: w136 -> [_ w229]
          tunnel: w135 -> [_ w228]
          frame False {
            n236 = case shown="True" w211 {
              tunnel: ["" w219] -> w205
              tunnel: w209 -> [_ w217]
              tunnel: w208 -> [_ w218]
              tunnel: "Save data 2 channels" -> [_ w216]
              tunnel: w207 -> [_ w215]
              tunnel: w206 -> [_ w214]
              frame False {
              }
              frame True {
                n237 = case shown="True" w216 {
                  tunnel: ["" w225] -> w219
                  tunnel: w217 -> [_ w224]
                  tunnel: w218 -> [_ w223]
                  tunnel: w215 -> [_ w222]
                  tunnel: w214 -> [_ w221]
                  frame False {
                  }
                  frame True {
                    n238 = Build Array(w224, w223, w222, w221) -> (w227:dbl[])
                    n239 = Array To Spreadsheet String(array=w227, 3:"%.3f") -> (spreadsheet string=w225:string)  [unwired: 1 out]
                  }
                }
              }
            }
          }
          frame True {
            n240 = case shown="True" w234 {
              tunnel: ["" w244] -> w232
              tunnel: w236 -> [_ w242]
              tunnel: w235 -> [_ w243]
              tunnel: "Save data 1 channel" -> [_ w241]
              tunnel: w230 -> [_ w240]
              tunnel: w229 -> [_ w239]
              tunnel: w228 -> [_ w238]
              frame False {
              }
              frame True {
                n241 = case shown="True" w241 {
                  tunnel: ["" w251] -> w244
                  tunnel: w242 -> [_ w249]
                  tunnel: w243 -> [_ w248]
                  tunnel: w240 -> [_ w250]
                  tunnel: w239 -> [_ w247]
                  tunnel: w238 -> [_ w246]
                  frame False {
                  }
                  frame True {
                    n242 = Build Array(w249, w248, w250, w247, w246) -> (w253:dbl[])
                    n243 = Array To Spreadsheet String(array=w253, 3:"%.3f") -> (spreadsheet string=w251:string)  [unwired: 1 out]
                  }
                }
              }
            }
          }
        }
      }
    }
    n244 = Write to Text File(file (use dialog)=w51, text=w46, error in=w50) -> (refnum out=w48:refnum<file>, error out=w49:errorcluster)  [unwired: 1 in, 1 out]
    n245 = Write to Text File(file (use dialog)=w57, text=w56, error in=w58) -> (refnum out=w59:refnum<file>, error out=w60:errorcluster)  [unwired: 1 in, 1 out]
    n246 = Write to Text File(file (use dialog)=w55, text=w47, error in=w53) -> (refnum out=w54:refnum<file>, error out=w52:errorcluster)  [unwired: 1 in, 1 out]
    "Numeric" <- w45
  }
  n247 = Close File(refnum=w22, error in=w23) -> (error out=w26:errorcluster)  [unwired: 1 out]
  n248 = Close File(refnum=w4, error in=w3) -> (error out=w10:errorcluster)  [unwired: 1 out]
  n249 = Close File(refnum=w2, error in=w1) -> (error out=w9:errorcluster)  [unwired: 1 out]
  n250 = local read "iterationsIM"() -> (→"iterationsIM":dbl)
  n251 = call <vilib>:"Simple Error Handler.vi"("error in (no error)"=w26) -> ()  [unwired: 1 in, 8 out]
  n252 = call <vilib>:"Simple Error Handler.vi"("error in (no error)"=w10) -> ()  [unwired: 1 in, 8 out]
  n253 = call <vilib>:"Simple Error Handler.vi"("error in (no error)"=w9) -> ()  [unwired: 1 in, 8 out]
  n254 = call <instrlib>:"niUSRP Close Session.vi"("session handle"=w36, "error in (no error)"=w37) -> ()  [unwired: 13 in, 1 out]
  "No. Bits LP - CH0" <- w33
  "No. Bits - CH1" <- w33
  "No. Bits HP - CH0" <- w33
